vi "Obtain Events.vi"(8 "error in (no error)":errorcluster caption="错误输入（无错误）", 10 "Create New?(F)":bool) -> (0 "error out":errorcluster caption="错误输出", 2 "helper loop data":T1)   [LabVIEW 2025, in "XButton.lvlib" / "button3.xctl"]
uses:
  button3.xctl
  helper loop Events.ctl
  move event.ctl
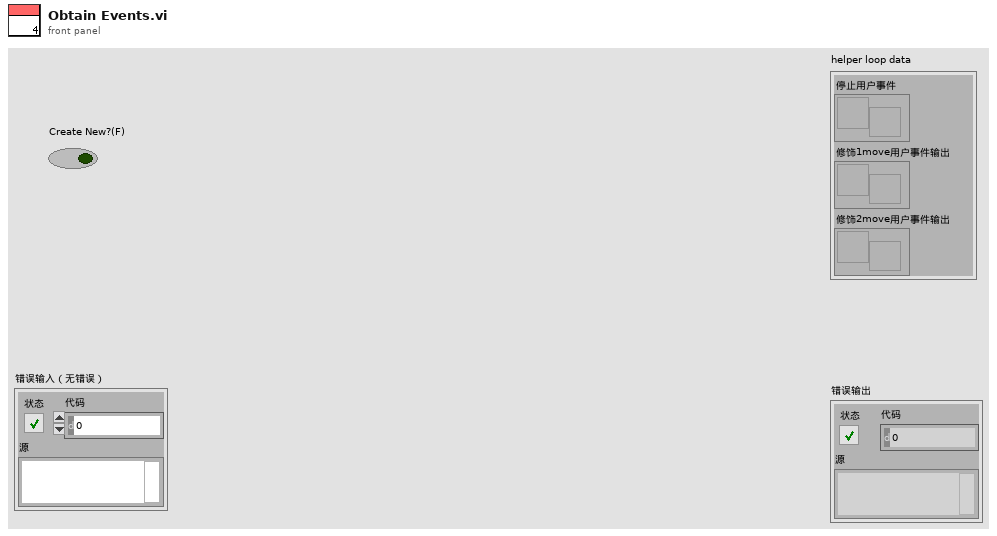
[diagram p1: front panel]
types:
  T1 = typedef "XButton.lvlib/button3.xctl/helper loop Events.ctl" = cluster{"停止用户事件":refnum<user-event>, "修饰1move用户事件输出":refnum<user-event>, "修饰2move用户事件输出":refnum<user-event>}
  T2 = typedef "XButton.lvlib/button3.xctl/move event.ctl" = cluster{"Decor引用句柄":refnum<vi>, "b":dbl, "c":dbl, "动效风格":enum16{"风格一", "风格二", "风格三", "风格四"}, "方向(T:离开/F:进入)":bool}
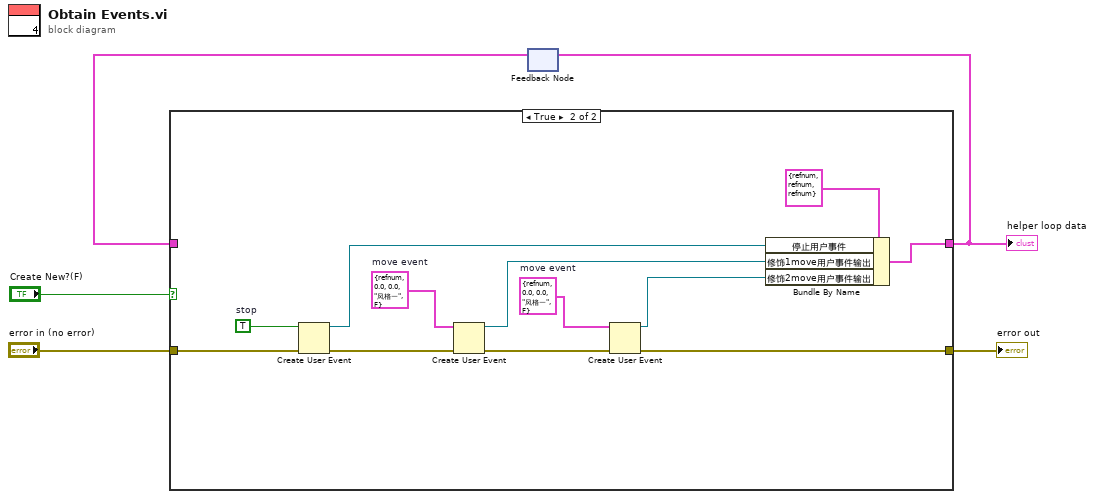
[diagram p0: block diagram]
diagram:
  n1 = feedback #1() -> (w4:T1)  [unwired: 1 in]
  n2 = case shown="True" "Create New?(F)" {
    tunnel: w4 -> [w7 _]
    tunnel: [w7 w18] -> w3
    tunnel: "error in (no error)" -> [w6 w15]
    tunnel: [w6 w10] -> w1
    frame False {
    }
    frame True {
      w9 = T2 {"Decor引用句柄"=refnum, "b"=0.0, "c"=0.0, "动效风格"=enum."风格一", "方向(T:离开/F:进入)"=FALSE}  # move event
      w14 = T2 {"Decor引用句柄"=refnum, "b"=0.0, "c"=0.0, "动效风格"=enum."风格一", "方向(T:离开/F:进入)"=FALSE}  # move event
      w17 = TRUE  # stop
      n3 = Create User Event(user event datatype=w17, error in=w15) -> (user event=w16:refnum<user-event>, error out=w13:errorcluster)
      n4 = Create User Event(user event datatype=w14, error in=w13) -> (user event=w12:refnum<user-event>, error out=w11:errorcluster)
      n5 = Create User Event(user event datatype=w9, error in=w11) -> (user event=w8:refnum<user-event>, error out=w10:errorcluster)
      n6 = Bundle By Name(cluster=T1 {"停止用户事件"=refnum, "修饰1move用户事件输出"=refnum, "修饰2move用户事件输出"=refnum} ("helper loop data"), "停止用户事件"=w16, "修饰1move用户事件输出"=w12, "修饰2move用户事件输出"=w8) -> (w18:T1)
    }
  }
  "helper loop data" <- w3
  "error out" <- w1
  n7 = feedback-in #1(w3) -> ()
